vi "Check and Download Bitfile.vi"(8 "error in":errorcluster) -> (0 "error out":errorcluster)   [LabVIEW 2020, in "SEECD System Explorer.lvlib"]
uses:
  SEECD System Explorer.lvlib
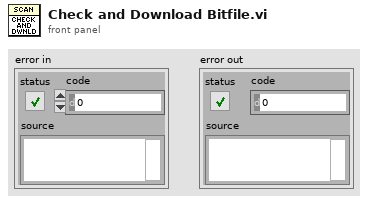
[diagram p1: front panel]
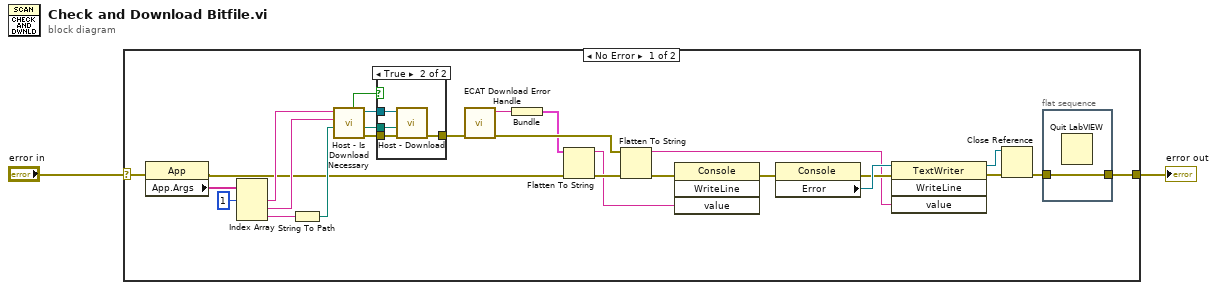
[diagram p0: block diagram]
diagram:
  n1 = case shown="No Error" "error in" {
    selector: "error in" -> [w28 w36]
    tunnel: [w26 w36] -> w1
    frame No Error {
      n2 = property class="App"(error in=w28) -> (error out=w6:errorcluster, "App.Args"=w29:string[])  [unwired: 1 in, 1 out]
      n3 = Index Array(array=w29, index #1=1 ("index")) -> (element #1=w20:string, element #2=w19:string, element #3=w25:string)  [unwired: 2 in]
      n4 = String To Path(string=w25) -> (path=w18:path)
      n5 = call "Host - Is Download Necessary.vi"("bitfile path in"=w18, "Target IP Address in"=w19, "Slave Ref in"=w20) -> ("error out"=w23:errorcluster, "bitfile path out"=w22:path, "Slave Ref out"=w21:refnum<k21>, "is download necessary?"=w24:bool)  [unwired: 4 in, 1 out]
      n6 = case shown="True" w24 {
        tunnel: w23 -> [w31 w35]
        tunnel: w22 -> [_ w34]
        tunnel: w21 -> [_ w33]
        tunnel: [w31 w32] -> w11
        frame False {
        }
        frame True {
          n7 = call "Host - Download.vi"("Error In (no error)"=w35, "bitfile path in"=w34, "Slave Ref in"=w33) -> ("error out"=w32:errorcluster)  [unwired: 6 in, 2 out]
        }
      }
      n8 = call "ECAT Download Error Handle.vi"("error in"=w11) -> ("error out"=w10:errorcluster, "Message output"=w5:string)  [unwired: 9 in]
      n9 = Bundle("Message output"=w5) -> (w4:cluster{"Message output":string})  [unwired: 1 in]
      n10 = Flatten To String(anything=w4, error in (no error)=w6) -> (data string=w3:string, error out=w7:errorcluster)  [unwired: 2 in, 1 out]
      n11 = Flatten To String(anything=w10, error in (no error)=w7) -> (data string=w13:string, error out=w8:errorcluster)  [unwired: 2 in, 1 out]
      n12 = invoke class="Console" method="WriteLine"(error in=w8, "value"=w3) -> (error out=w9:errorcluster)  [unwired: 2 in, 3 out]
      n13 = property class="Console"(error in=w9) -> (error out=w15:errorcluster, "Error"=w17:refnum<k24>)  [unwired: 1 in, 1 out]
      n14 = invoke class="TextWriter" method="WriteLine"(reference=w17, error in=w15, "value"=w13) -> (reference out=w12:refnum<k24>, error out=w16:errorcluster)  [unwired: 1 in, 2 out]
      n15 = Close Reference(reference=w12, error in (no error)=w16) -> (error out=w14:errorcluster)
      n16 = flat-sequence {
        tunnel: w14 -> [w30]
        tunnel: [w30] -> w26
        frame #0 {
          n17 = Quit LabVIEW() -> ()  [unwired: 1 in]
        }
      }
    }
    frame Error {
    }
  }
  "error out" <- w1
